vi "Watchdog Start.vi"(4 "error in (no error)":errorcluster, 7 "watchdogID in":u64 format="%.0x") -> (0 "error out":errorcluster, 3 "watchdogID out":u64 format="%.0x")   [LabVIEW 2025]
doc: "<p>Restarts the countdown of the <a href=\"nihelplauncher://docs/csh?context=lvrt_lvrtconcepts_rt_watchdog\">watchdog timer</a> if the watchdog object is running or expired.</p>"
uses:
  niwd4c.dll
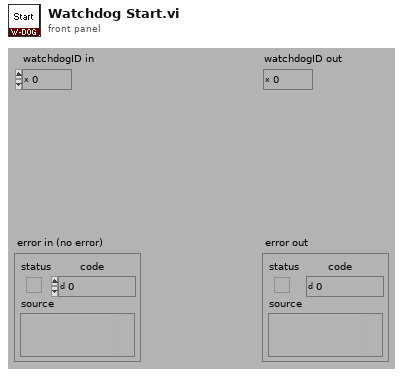
[diagram p1: front panel]
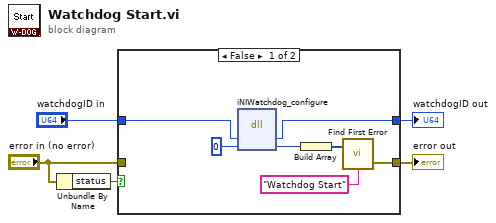
[diagram p0: block diagram]
diagram:
  n1 = Unbundle By Name("error in (no error)") -> ("status"=w5:bool)
  n2 = case shown="False" w5 {
    tunnel: [w8 w13] -> w2
    tunnel: [w11 w14] -> w3
    tunnel: "error in (no error)" -> [_ w14]
    tunnel: "watchdogID in" -> [w6 w13]
    frame False {
      n3 = dll-call lib="niwd4c.*" fn="iNIWatchdog_configure" label="Configure"("wd"=w6, "status"=0) -> ("wd"=w8:u64, "status"=w9:i32)  [unwired: 4 in, 2 out]
      n4 = Build Array(w9) -> (w12:i32[])
      n5 = call <vilib>:"Find First Error.vi"("source messages"="Watchdog Start", "error codes"=w12) -> ("error out"=w11:errorcluster)  [unwired: 2 in, 1 out]
    }
    frame True {
    }
  }
  "error out" <- w3
  "watchdogID out" <- w2
